vi "Convert XNET CAN Status.vi"(11 "CAN comm State":T4 {"fault code" format="%08x"; "last error" items=["None", "Stuff", "Form", "Ack", "Bit1", "Bit0", "CRC"]; "communication state" items=["Error Active", "Error Passive", "Bus Off", "Init"]}) -> (3 "CAN Status":T1)   [LabVIEW 2021, in "XNET CAN RW.lvclass"]
uses:
  XNET CAN RW.lvclass
  XNET CAN RW.lvclass/XNET CAN RW.ctl
  <vilib>/CIF Foundation/CIF CAN RW Core/typedef/Last Error.ctl
  <vilib>/CIF Foundation/CIF CAN RW Core/CAN_RW_CORE.lvclass
  <vilib>/CIF Foundation/CIF CAN RW Core/typedef/Communication State.ctl
  <vilib>/CIF Foundation/CIF CAN RW Core/typedef/CAN Status.ctl
  <vilib>/xnet/xnet.llb/XNET CAN Comm State.ctl
  <vilib>/xnet/xnet.llb/XNET CAN Last Err.ctl
  <vilib>/xnet/xnet.llb/XNET CAN Comm.ctl
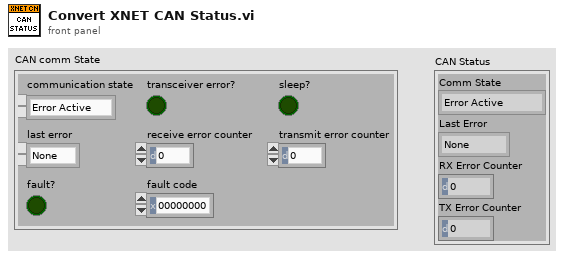
[diagram p1: front panel]
types:
  T1 = typedef "CAN_RW_CORE.lvclass/CAN Status.ctl" = cluster{"Comm State":T2, "Last Error":T3, "RX Error Counter":u8, "TX Error Counter":u8}
  T2 = typedef "CAN_RW_CORE.lvclass/Communication State.ctl" = enum16{"Error Active", "Error Passive", "Bus Off"}
  T3 = typedef "CAN_RW_CORE.lvclass/Last Error.ctl" = enum16{"None", "Stuff", "Form", "Ack", "Bit1", "Bit0", "CRC", "Unknown"}
  T4 = typedef "XNET CAN Comm.ctl" = cluster{"fault code":i32, "fault?":bool, "communication state":T5, "last error":T6, "receive error counter":u8, "transmit error counter":u8, "transceiver error?":bool, "sleep?":bool}
  T5 = typedef "XNET CAN Comm State.ctl" = u8
  T6 = typedef "XNET CAN Last Err.ctl" = u8
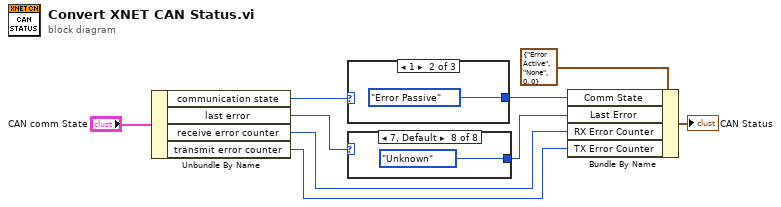
[diagram p0: block diagram]
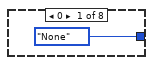
[diagram p2: hidden frame]
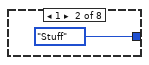
[diagram p3: hidden frame]
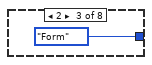
[diagram p4: hidden frame]
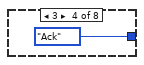
[diagram p5: hidden frame]
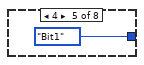
[diagram p6: hidden frame]
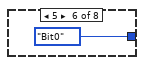
[diagram p7: hidden frame]
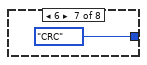
[diagram p8: hidden frame]
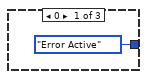
[diagram p9: hidden frame]
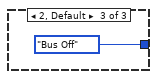
[diagram p10: hidden frame]
diagram:
  n1 = Unbundle By Name("CAN comm State") -> ("communication state"=w6:T5, "last error"=w4:T6, "receive error counter"=w2:u8, "transmit error counter"=w3:u8)
  n2 = case shown="1" w6 {
    tunnel: [Communication_State."Error Active" ("Comm State") Communication_State."Error Passive" ("Comm State") Communication_State."Bus Off" ("Comm State")] -> w7
    frame 0 {
    }
    frame 1 {
    }
    frame 2, Default {
    }
  }
  n3 = case shown="7, Default" w4 {
    tunnel: [Last_Error."None" ("Last Error") Last_Error."Stuff" ("Last Error") Last_Error."Form" ("Last Error") Last_Error."Ack" ("Last Error") Last_Error."Bit1" ("Last Error") Last_Error."Bit0" ("Last Error") Last_Error."CRC" ("Last Error") Last_Error."Unknown" ("Last Error")] -> w5
    frame 0 {
    }
    frame 1 {
    }
    frame 2 {
    }
    frame 3 {
    }
    frame 4 {
    }
    frame 5 {
    }
    frame 6 {
    }
    frame 7, Default {
    }
  }
  n4 = Bundle By Name(cluster=T1 {"Comm State"=enum."Error Active", "Last Error"=enum."None", "RX Error Counter"=0, "TX Error Counter"=0} ("CAN Status"), "Comm State"=w7, "Last Error"=w5, "RX Error Counter"=w2, "TX Error Counter"=w3) -> (→"CAN Status":T1)
